vi "VM Spy - Dialog - Alias Info.vi"(10 "var name":string, 11 "vc handle":T1=-1) -> (0 "cancel out":bool)   [LabVIEW 2021]
doc: "::: CalcExpress Toolkit :::\nCopyright (c) 2000-2026 Konstantin Shifershteyn. All rights reserved."
uses:
  vi.lib/addons/CalcExpress/cetypes.llb/VarMan Variable Context Handle.ctl
panel:
  in  "cancel":bool caption="Cancel"
  in  "dispose":bool caption="Dispose"
  out "Context":string
  out "Variable name":string
  in  "assign":bool caption="Assign/Rename"
  in  "Alias":string
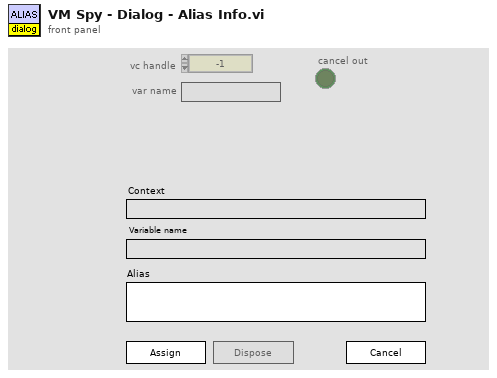
[diagram p1: front panel]
types:
  T1 = typedef "VarMan Variable Context Handle.ctl" = i32
  T2 = typedef "eventvkey.ctl" = enum16{"ASCII", "Enter", "Return", "Shift", "Ctrl", "Alt", "Cmd", "Opt", "Caps", "NumLock", "Clear", "Break", "Up", "Down", "Left", "Right", "Insert", "Delete", "Home", "End", "PageUp", "PageDown", "Escape", "Help", "Pause", "ScrollLock", "F1", "F2", "F3", "F4", "F5", "F6", "F7", "F8", "F9", "F10", "F11", "F12", "F13", "F14", "F15", "F16", "F17", "F18", "F19", "F20", "F21", "F22", "F23", "F24", "Play", "VolumeUp", "VolumeDown", "Mute", "Two Byte Char"}
  T3 = cluster{"Shift":bool, "Ctrl":bool, "Alt":bool, "Cmd":bool, "Opt":bool}
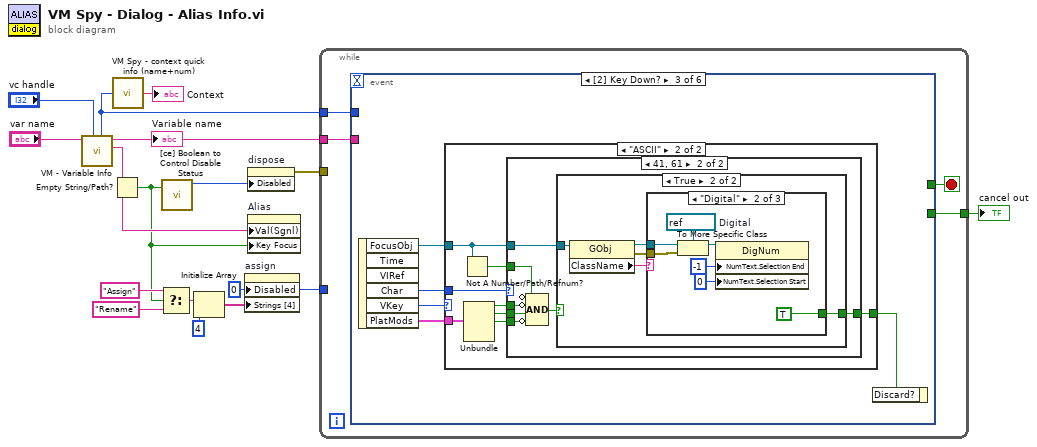
[diagram p0: block diagram]
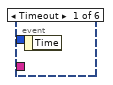
[diagram p2: hidden frame]
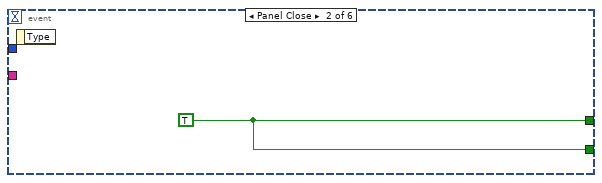
[diagram p3: hidden frame]
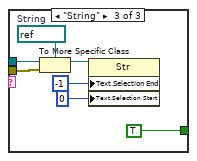
[diagram p8: hidden frame]
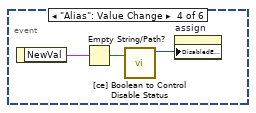
[diagram p9: hidden frame]
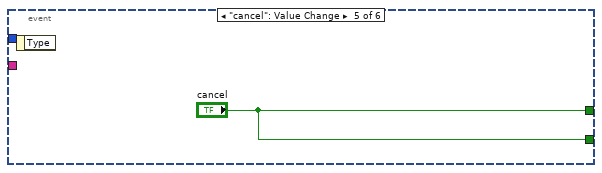
[diagram p10: hidden frame]
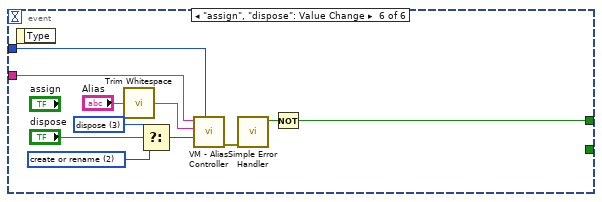
[diagram p11: hidden frame]
diagram:
  w5 = u8 0 ("Disabled")
  n1 = call "VM - Variable Info.vi"("VC Handle"="vc handle", "name_spec"="var name") -> ("alias"=w4:string, "var name"=w12:string, "var VC Handle"=w11:T1)  [unwired: 4 in, 3 out]
  "Variable name" <- w12
  n2 = Empty String/Path?(string/path=w4) -> (empty?=w3:bool)
  n3 = call "VM Spy - context quick info (name+num).vi"("handle"=w11) -> ("context info"=→"Context":string)  [unwired: 4 in]
  n4 = Select(t="Assign", s=w3, f="Rename") -> (s? t:f=w8:string)
  n5 = call "[ce] Boolean to Control Disable Status.vi"("Status in"=w3) -> ("Control Disable if True"=w2:u8)  [unwired: 3 in, 1 out]
  n6 = Initialize Array(w8, 4 ("dimension size")) -> (w6:string[])
  n7 = property on="assign" class="Bool"("Disabled"=w5, "Strings [4]"=w6) -> ()  [unwired: 2 in, 2 out]
  n8 = property on="dispose" class="Bool"("Disabled"=w2) -> (error out=w1:errorcluster)  [unwired: 2 in, 1 out]
  n9 = property on="Alias" class="Str"("Val(Sgnl)"=w4, "Key Focus"=w3) -> ()  [unwired: 2 in, 2 out]
  n10 = while {
    tunnel: w12 -> [w19]
    tunnel: [w18] -> w13
    tunnel: w11 -> [w17]
    tunnel: w5 -> [_]
    tunnel: w1 -> [_]
    stop <- w20 stop-if-true
    n11 = event shown="[2] Key Down?" {
      selector: _ -> [_ _ _ _ _ _]
      dyn-events: _ -> [_ _ _ _ _ _]
      timeout: _ -> [_ _ _ _ _ _]
      tunnel: [_ w21 _ _ "cancel" w68] -> w20
      tunnel: w19 -> [_ _ _ _ _ w67]
      tunnel: [_ w21 _ _ "cancel" _] -> w18
      tunnel: w17 -> [_ _ _ _ _ w66]
      event Timeout {
        n12 = event-data() -> ()  [unwired: 1 in, 1 out]
      }
      event Panel Close {
        w21 = TRUE
        n13 = event-data() -> ()  [unwired: 1 in, 1 out]
      }
      event Key Down? {
        n14 = event-data() -> ("FocusObj"=w24:refnum<vi>, "Char"=w25:i16, "VKey"=w26:T2, "PlatMods"=w23:T3)  [unwired: 1 in, 2 out]
        n15 = case shown="\"ASCII\"" w26 {
          tunnel: w23 -> [_ w34]
          tunnel: [_ w28] -> w22
          tunnel: w25 -> [_ w30]
          tunnel: w24 -> [_ w29]
          frame Default {
          }
          frame "ASCII" {
            n16 = Not A Number/Path/Refnum?(number/path/refnum=w29) -> (NaN/Path/Refnum?=w27:bool)
            n17 = Unbundle(w34) -> ("Shift"=w33:bool, "Ctrl"=w32:bool, "Alt"=w31:bool)  [unwired: 2 out]
            n18 = case shown="41, 61" w30 {
              tunnel: w33 -> [_ w41]
              tunnel: w32 -> [_ w40]
              tunnel: w31 -> [_ w39]
              tunnel: w29 -> [_ w37]
              tunnel: [_ w36] -> w28
              tunnel: w27 -> [_ w35]
              frame Default {
              }
              frame 65, 97 {
                n19 = Compound Arithmetic op=AND(invert w35, invert w41, w40, invert w39) -> (w38:bool)
                n20 = case shown="True" w38 {
                  tunnel: w37 -> [_ w46]
                  tunnel: [_ w44] -> w36
                  frame False {
                  }
                  frame True {
                    n21 = property class="GObj"(reference=w46) -> (reference out=w43:refnum<vi>, error out=w42:errorcluster, "ClassName"=w45:string)  [unwired: 1 in]
                    n22 = case shown="\"Digital\"" w45 {
                      tunnel: [_ TRUE TRUE] -> w44
                      tunnel: w43 -> [_ w51 w58]
                      tunnel: w42 -> [_ w50 w57]
                      frame Default {
                      }
                      frame "Digital" {
                        w52 = refnum<vi> refnum  # Digital
                        n23 = To More Specific Class(target class=w52, reference=w51, error in=w50) -> (specific class reference=w49:refnum<vi>)  [unwired: 1 out]
                        n24 = property class="DigNum"(reference=w49, "NumText.Selection End"=-1 ("Numeric Text.Selection:End"), "NumText.Selection Start"=u32 0 ("Numeric Text.Selection:Start")) -> ()  [unwired: 1 in, 2 out]
                      }
                      frame "String" {
                        w59 = refnum<vi> refnum  # String
                        n25 = To More Specific Class(target class=w59, reference=w58, error in=w57) -> (specific class reference=w56:refnum<vi>)  [unwired: 1 out]
                        n26 = property class="Str"(reference=w56, "Text.Selection End"=-1 ("Numeric Text.Selection:End"), "Text.Selection Start"=u32 0 ("Numeric Text.Selection:Start")) -> ()  [unwired: 1 in, 2 out]
                      }
                    }
                  }
                }
              }
            }
          }
        }
        n27 = event-data("Discard?"=w22) -> ()  [unwired: 1 in, 1 out]
      }
      event "Alias": Value Change {
        n28 = event-data() -> ("NewVal"=w63:string)  [unwired: 1 in]
        n29 = Empty String/Path?(string/path=w63) -> (empty?=w62:bool)
        n30 = call "[ce] Boolean to Control Disable Status.vi"("Status in"=w62) -> ("Control Disable if True"=w61:u8)  [unwired: 3 in, 1 out]
        n31 = property on="assign" class="Bool"("DisabledEnum"=w61) -> ()  [unwired: 2 in, 2 out]
      }
      event "cancel": Value Change {
        n32 = event-data() -> ()  [unwired: 1 in, 1 out]
      }
      event "assign", "dispose": Value Change {
        w73 = u32 2 items=["nop", "create", "create or rename", "dispose"] ("action")
        w72 = u32 3 items=["nop", "create", "create or rename", "dispose"] ("action")
        n33 = event-data() -> ()  [unwired: 1 in, 1 out]
        n34 = call <vilib>:"Trim Whitespace.vi"("string"="Alias") -> ("trimmed string"=w65:string)  [unwired: 1 in]
        n35 = Select(t=w72, s="dispose", f=w73) -> (s? t:f=w71:u32)
        n36 = call "VM - Alias Controller.vi"("VC Handle"=w66, "action"=w71, "alias"=w65, "name_spec"=w67) -> ("error out"=w75:errorcluster)  [unwired: 4 in, 3 out]
        n37 = call <vilib>:"Simple Error Handler.vi"("error in (no error)"=w75) -> ("error?"=w69:bool)  [unwired: 4 in, 4 out]
        n38 = Not(x=w69) -> (.not. x?=w68:bool)
      }
    }
  }
  "cancel out" <- w13
